vi "Open Vi by path.vi"(6 "Execution:Run When Opened":bool, 8 "error in (no error)":errorcluster, 11 "vi path":path) -> (0 "error IO":errorcluster, 3 "Error?":bool)   [LabVIEW 2020]
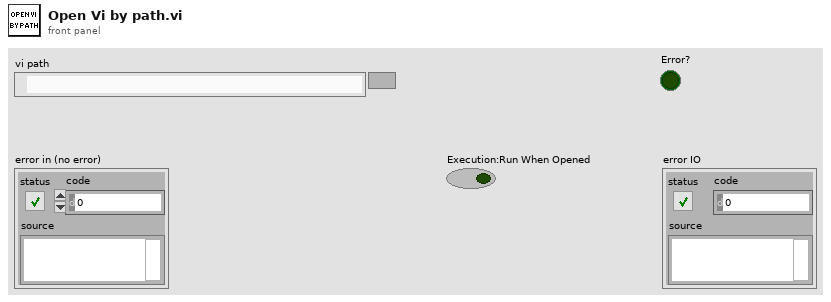
[diagram p1: front panel]
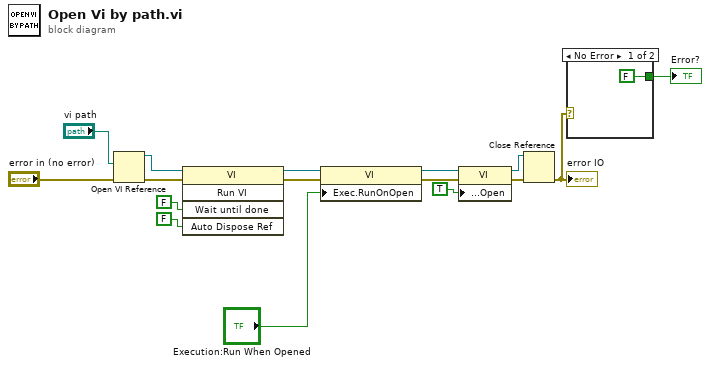
[diagram p0: block diagram]
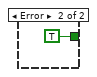
[diagram p2: hidden frame]
diagram:
  n1 = Open VI Reference(vi path="vi path", error in (no error)="error in (no error)") -> (vi reference=w10:refnum<vi>, error out=w11:errorcluster)  [unwired: 4 in]
  n2 = invoke class="VI" method="Run VI"(reference=w10, error in=w11, "Wait until done"=FALSE ("Wait Until Done"), "Auto Dispose Ref"=FALSE ("Auto Dispose Reference")) -> (reference out=w5:refnum<vi>, error out=w4:errorcluster)  [unwired: 1 in, 3 out]
  n3 = property class="VI"(reference=w5, error in=w4, "Exec.RunOnOpen"="Execution:Run When Opened") -> (reference out=w3:refnum<vi>, error out=w2:errorcluster)
  n4 = property class="VI"(reference=w3, error in=w2, "Front Panel Window:Open"=TRUE) -> (reference out=w8:refnum<vi>, error out=w7:errorcluster)
  n5 = Close Reference(reference=w8, error in (no error)=w7) -> (error out=w6:errorcluster)
  "error IO" <- w6
  n6 = case shown="No Error" w6 {
    tunnel: [FALSE ("Error?") TRUE ("Error?")] -> w12
    frame No Error {
    }
    frame Error {
    }
  }
  "Error?" <- w12
